vi "FuncVI2-SearchPath.vi"(4 "CSE RefNum":T1, 5 "InstanceRef":T3, 9 "arg list":T2[](array[typedef]) {"num" format="%.2f"}) -> (0 "error out":bool, 3 "result":T2 {"num" format="%.2f"})   [LabVIEW 2021]
doc: "::: CalcExpress Toolkit :::\nCopyright (c) 2000-2026 Konstantin Shifershteyn. All rights reserved."
uses:
  cetypes.llb/CalcExpress Function Argument Info.ctl
  cetypes.llb/CalcExpress Instance RefNum.ctl
  cse.llb/CSE Instance RefNum.ctl
panel:
  in  "max arg num":i32=1000
  in  "min arg num":i32
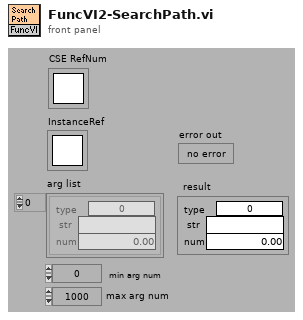
[diagram p1: front panel]
types:
  T1 = typedef "CSE Instance RefNum.ctl" = refnum<k1>
  T2 = typedef "CalcExpress Function Argument Info.ctl" = cluster{"type":u32, "str":string, "num":dbl}
  T3 = typedef "CalcExpress Instance RefNum.ctl" = refnum<k1>
  T4 = enum32{"String", "DBL Number", "identifier", "1D Array of DBL", "2D Array of DBL", "CDB Number", "1D Array of CDB", "2D Array of CDB", "1D Array of String", "2D Array of String", "Unknown data type"}
  T5 = cluster{"type: use this constant to specify a predefined type code":enum32{"String", "DBL Number", "identifier", "1D Array of DBL", "2D Array of DBL", "CDB Number", "1D Array of CDB", "2D Array of CDB", "1D Array of String", "2D Array of String", "Unknown data type"}, "data string":string, dbl}
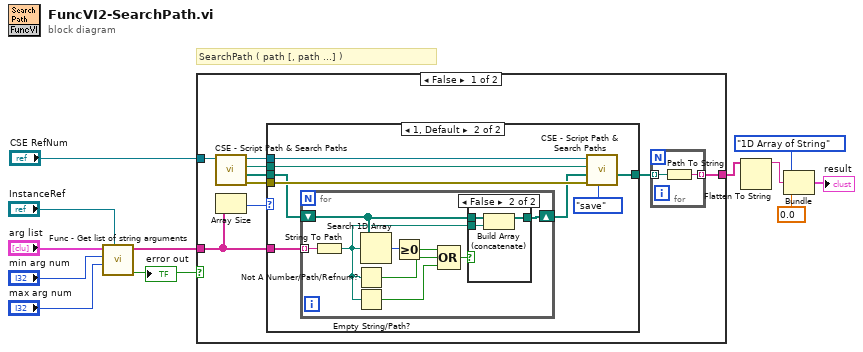
[diagram p0: block diagram]
diagram:
  # "SearchPath ( path [, path ...] )"
  n1 = call "Func - Get list of string arguments.vi"("InstanceRef"="InstanceRef", "max arg num"="max arg num", "min arg num"="min arg num", "arg list"="arg list") -> ("error out"=w2:bool, "val list"=w8:string[])  [unwired: 4 in]
  "error out" <- w2
  n2 = case shown="False" w2 {
    tunnel: w8 -> [w16 _]
    tunnel: [w14 _] -> w5
    tunnel: "CSE RefNum" -> [w13 _]
    frame False {
      n3 = call "CSE - Script Path & Search Paths.vi"("CSE RefNum"=w13) -> ("error out"=w21:errorcluster, "search paths out"=w18:path[], "script file path out"=w20:path, "dup CSE RefNum"=w19:T1)  [unwired: 7 in]
      n4 = Array Size(array=w16) -> (size(s)=w17:i32)
      n5 = case shown="1, Default" w17 {
        tunnel: w21 -> [_ w32]
        tunnel: w20 -> [_ w31]
        tunnel: w19 -> [_ w30]
        tunnel: w16 -> [_ w29]
        tunnel: w18 -> [w24 w26]
        tunnel: [w24 w28] -> w15
        frame 0 {
        }
        frame 1, Default {
          n6 = for {
            tunnel: w29 -> [w41] mode=indexing
            shift-right: [w39] -> w25
            shift-left: w26 -> [w40]
            n7 = String To Path(string=w41) -> (path=w38:path)
            n8 = Not A Number/Path/Refnum?(number/path/refnum=w38) -> (NaN/Path/Refnum?=w35:bool)
            n9 = Empty String/Path?(string/path=w38) -> (empty?=w34:bool)
            n10 = Search 1D Array(1D array=w40, element=w38) -> (index of element=w37:i32)  [unwired: 1 in]
            n11 = Greater Or Equal To 0?(x=w37) -> (x >= 0?=w36:bool)
            n12 = Compound Arithmetic op=OR(w36, w35, w34) -> (w33:bool)
            n13 = case shown="False" w33 {
              tunnel: w40 -> [w42 w45]
              tunnel: [w42 w44] -> w39
              tunnel: w38 -> [_ w43]
              frame True {
              }
              frame False {
                n14 = Build Array (concatenate)(w45, w43) -> (w44:path[])
              }
            }
          }
          n15 = call "CSE - Script Path & Search Paths.vi"("action"=enum32{"get", "save"}."save", "error in"=w32, "search paths"=w25, "script file path"=w31, "CSE RefNum"=w30) -> ("search paths out"=w28:path[])  [unwired: 3 in, 3 out]
        }
      }
      n16 = for {
        tunnel: w15 -> [w23] mode=indexing
        tunnel: [w22] -> w14 mode=indexing
        n17 = Path To String(path=w23) -> (string=w22:string)
      }
    }
    frame True {
    }
  }
  n18 = Flatten To String(anything=w5) -> (data string=w4:string)  [unwired: 3 in, 2 out]
  n19 = Bundle("type: use this constant to specify a predefined type code"=T4."1D Array of String", "data string"=w4, 0.0) -> (→"result":T5)  [unwired: 1 in]
